vi "DAC Run.vi"(8 "error in":errorcluster, 11 "DAC DC Supply in":refnum<class "DAC DC Supply.lvclass">) -> (0 "error out":errorcluster, 3 "DAC DC Supply out":refnum<class "DAC DC Supply.lvclass">)   [LabVIEW 2019, in "DAC.lvlib" / "DAC DC Supply.lvclass"]
uses:
  DAC DC Supply.lvclass
  C:/Users/krio/Documents/LV_Projects/test-stand/App/DAC/DAC.lvclass
  DAC.lvclass/DAC.ctl
  Results/Results Method.ctl
  Results/HTS Results/HTS Results.lvclass
  DAC DC Supply.lvclass/DAC DC Supply.ctl
  DAC.lvclass
  Results/Results.lvlib
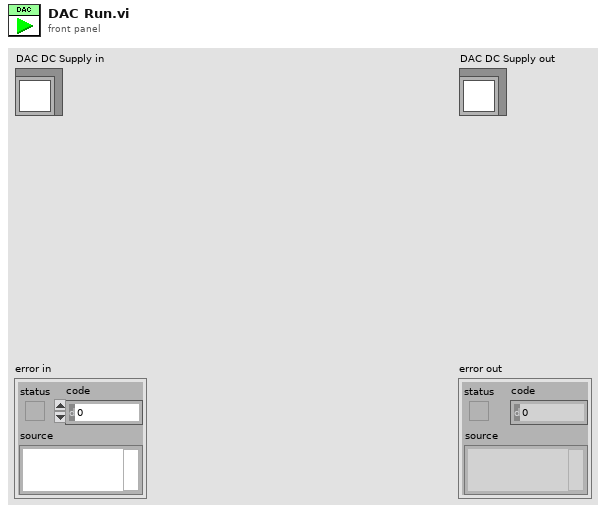
[diagram p1: front panel]
types:
  T1 = typedef "Results.lvlib/Results Method.ctl" = enum16{"Get", "Set"}
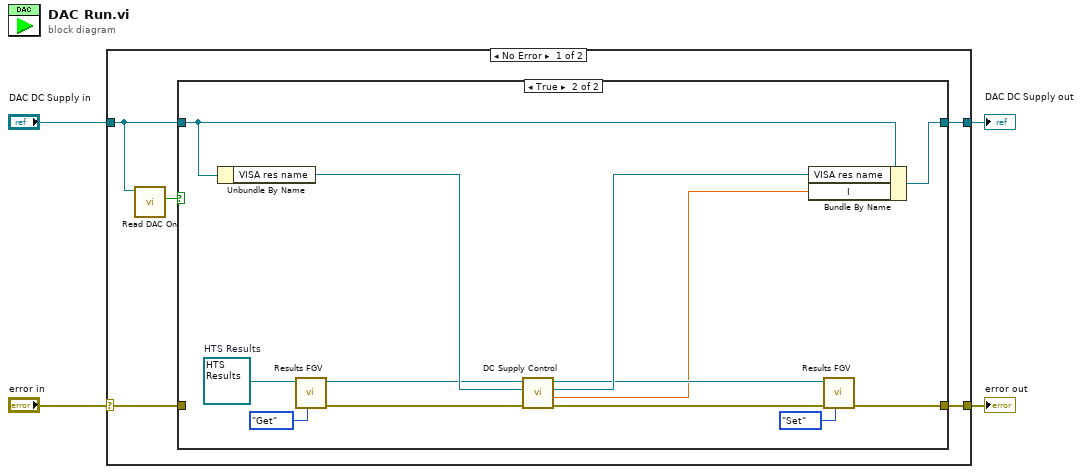
[diagram p0: block diagram]
diagram:
  n1 = case shown="No Error" "error in" {
    selector: "error in" -> [w7 w26]
    tunnel: [w6 w26] -> w2
    tunnel: [w8 w25] -> w1
    tunnel: "DAC DC Supply in" -> [w5 w25]
    frame No Error {
      n2 = call "Read DAC On.vi"("DAC in"=w5) -> ("DAC On"=w9:bool)  [unwired: 8 in, 2 out]
      n3 = case shown="True" w9 {
        tunnel: w5 -> [w11 w24]
        tunnel: [w11 w22] -> w8
        tunnel: w7 -> [w10 _]
        tunnel: [w10 w19] -> w6
        frame False {
        }
        frame True {
          w21 = refnum<class "HTS Results.lvclass"> refnum  # HTS Results
          n4 = Unbundle By Name(w24) -> ("VISA res name"=w18:refnum<visa-resource-name>)
          n5 = call-dynamic "Results FGV.vi"("Method"=Results_Method."Get", "HTS Results in"=w21) -> ("error out"=w14:errorcluster, "HTS Results out"=w16:refnum<class "HTS Results.lvclass">)  [unwired: 8 in]
          n6 = call "DC Supply Control.vi"("error in"=w14, "VISA res in"=w18, "HTS Results in"=w16) -> ("error out"=w13:errorcluster, "Supp I"=w12:dbl, "VISA res out"=w17:refnum<visa-resource-name>, "HTS Results out"=w15:refnum<class "HTS Results.lvclass">)  [unwired: 5 in]
          n7 = Bundle By Name(cluster=w24, "VISA res name"=w17, "I"=w12) -> (w22:refnum<class "DAC DC Supply.lvclass">)
          n8 = call-dynamic "Results FGV.vi"("Method"=Results_Method."Set", "error in"=w13, "HTS Results in"=w15) -> ("error out"=w19:errorcluster)  [unwired: 7 in, 1 out]
        }
      }
    }
    frame Error {
    }
  }
  "error out" <- w2
  "DAC DC Supply out" <- w1
